vi "Sim_Check_Completion.vi"(9 "State":T3=enum."CHARGING", 10 "Settings":T4={"UI Update Interval (ms)"=200, "Max dt (s)"=1.0, "Initial SOC (%)"=50.0, "Rest Voltage (V)"=12.0, "Ambient Temperature (degC)"=25.0, "Voltage Time Constant (s)"=5.0, "Current Time Constant (s)"=1.0, "Thermal Time Constant (s)"=120.0, "Heating Coefficient (degC/s per A^2)"=0.002, "SOC Speed Factor"=1.0, "Charge Complete SOC (%)"=100.0, "Discharge Complete SOC (%)"=0.0, "Max Voltage Limit (V)"=15.0, "Max Current Limit (A)"=10.0, "Max Temperature Limit (degC)"=45.0, "Max C-Rate (1/h)"=5.0, "Max Duration (min)"=600.0, "History Length (samples)"=3000, "Inject E-Stop"=FALSE, "Inject Overvoltage"=FALSE, "Inject Overcurrent"=FALSE, "Inject Overtemperature"=FALSE}, 11 "Sim Data in":T1) -> (2 "Done?":bool, 3 "Sim Data out":T1)   [LabVIEW 2019]
doc: "Completion check for CHARGING / DISCHARGING. Done when the SOC target is reached (charge: SOC at or above Charge Complete SOC; discharge: SOC at or below Discharge Complete SOC) or the setpoint duration has elapsed. CYCLE DEFINITION: a half-cycle counts only when its SOC target is reached; duration expiry does not count. When both halves are done (either order) Cycle Count increments once and both flags clear. Not done: data passes through unchanged."
uses:
  Sim_Data.ctl
  Test_State_Enum2.ctl
  Sim_Settings.ctl
  Sim_State_Enum.ctl
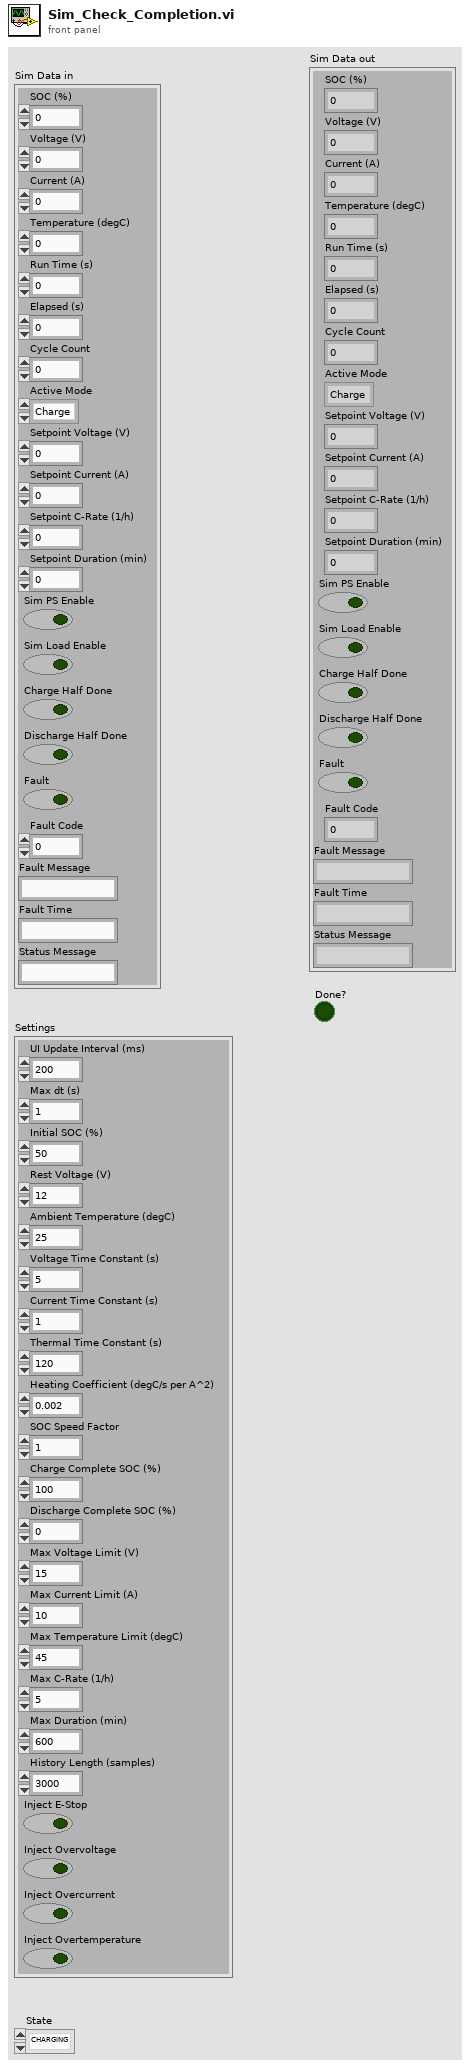
[diagram p1: front panel]
types:
  T1 = typedef "Sim_Data.ctl" = cluster{"SOC (%)":dbl, "Voltage (V)":dbl, "Current (A)":dbl, "Temperature (degC)":dbl, "Run Time (s)":dbl, "Elapsed (s)":dbl, "Cycle Count":u32, "Active Mode":T2, "Setpoint Voltage (V)":dbl, "Setpoint Current (A)":dbl, "Setpoint C-Rate (1/h)":dbl, "Setpoint Duration (min)":dbl, "Sim PS Enable":bool, "Sim Load Enable":bool, "Charge Half Done":bool, "Discharge Half Done":bool, "Fault":bool, "Fault Code":i32, "Fault Message":string, "Fault Time":string, "Status Message":string}
  T2 = typedef "Test_State_Enum2.ctl" = enum16{"Charge", "Discharge"}
  T3 = typedef "Sim_State_Enum.ctl" = enum16{"INIT", "IDLE", "CHARGING", "DISCHARGING", "STOPPED", "FAULT"}
  T4 = typedef "Sim_Settings.ctl" = cluster{"UI Update Interval (ms)":i32, "Max dt (s)":dbl, "Initial SOC (%)":dbl, "Rest Voltage (V)":dbl, "Ambient Temperature (degC)":dbl, "Voltage Time Constant (s)":dbl, "Current Time Constant (s)":dbl, "Thermal Time Constant (s)":dbl, "Heating Coefficient (degC/s per A^2)":dbl, "SOC Speed Factor":dbl, "Charge Complete SOC (%)":dbl, "Discharge Complete SOC (%)":dbl, "Max Voltage Limit (V)":dbl, "Max Current Limit (A)":dbl, "Max Temperature Limit (degC)":dbl, "Max C-Rate (1/h)":dbl, "Max Duration (min)":dbl, "History Length (samples)":i32, "Inject E-Stop":bool, "Inject Overvoltage":bool, "Inject Overcurrent":bool, "Inject Overtemperature":bool}
  T5 = enum16{"INIT", "IDLE", "CHARGING", "DISCHARGING", "STOPPED", "FAULT"}
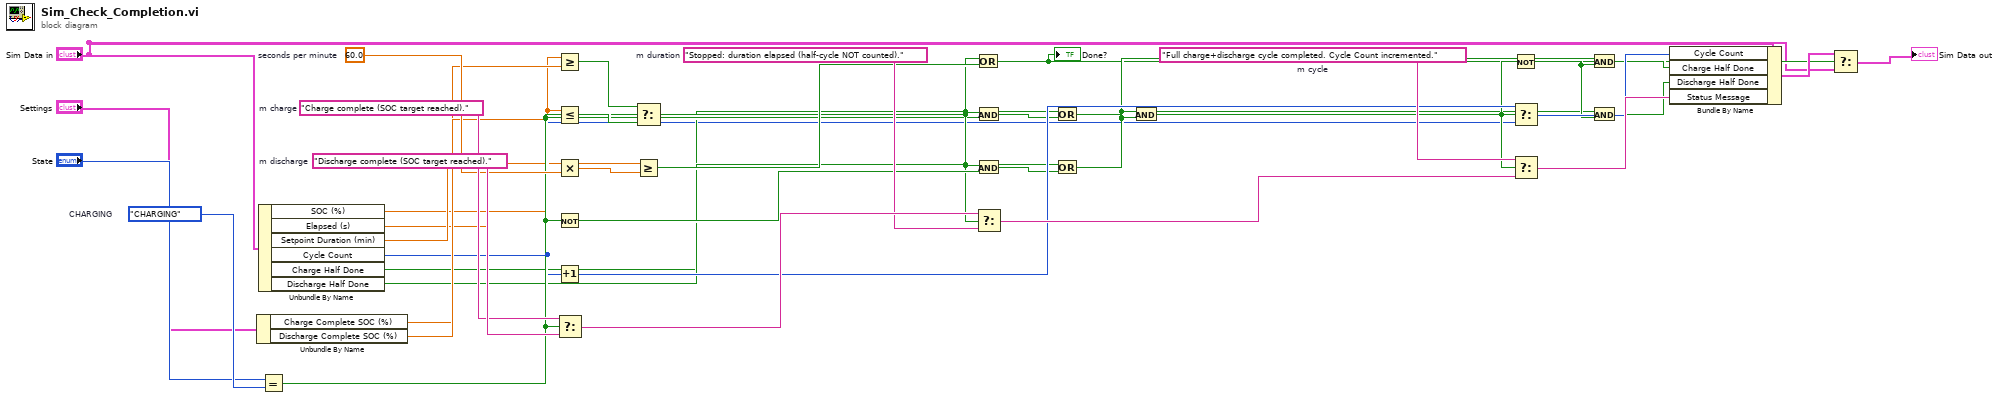
[diagram p0: block diagram]
diagram:
  w36 = "Full charge+discharge cycle completed. Cycle Count incremented."  # m cycle
  w35 = "Stopped: duration elapsed (half-cycle NOT counted)."  # m duration
  w34 = "Discharge complete (SOC target reached)."  # m discharge
  w33 = "Charge complete (SOC target reached)."  # m charge
  w19 = 60.0  # seconds per minute
  w14 = T5."CHARGING"  # CHARGING
  n1 = Unbundle By Name("Settings") -> ("Charge Complete SOC (%)"=w12:dbl, "Discharge Complete SOC (%)"=w13:dbl)
  n2 = Unbundle By Name("Sim Data in") -> ("SOC (%)"=w6:dbl, "Elapsed (s)"=w7:dbl, "Setpoint Duration (min)"=w8:dbl, "Cycle Count"=w9:u32, "Charge Half Done"=w10:bool, "Discharge Half Done"=w11:bool)
  n3 = Equal?(x="State", y=w14) -> (x = y?=w15:bool)
  n4 = Greater Or Equal?(x=w6, y=w12) -> (x >= y?=w16:bool)
  n5 = Less Or Equal?(x=w6, y=w13) -> (x <= y?=w17:bool)
  n6 = Multiply(x=w8, y=w19) -> (x*y=w20:dbl)
  n7 = Not(x=w15) -> (.not. x?=w22:bool)
  n8 = Increment(x=w9) -> (x+1=w31:u32)
  n9 = Select(t=w33, s=w15, f=w34) -> (s? t:f=w37:string)
  n10 = Select(t=w16, s=w15, f=w17) -> (s? t:f=w18:bool)
  n11 = Greater Or Equal?(x=w7, y=w20) -> (x >= y?=w21:bool)
  n12 = Or(x=w18, y=w21) -> (x .or. y?=w5:bool)
  "Done?" <- w5
  n13 = And(x=w18, y=w15) -> (x .and. y?=w23:bool)
  n14 = And(x=w18, y=w22) -> (x .and. y?=w24:bool)
  n15 = Select(t=w37, s=w18, f=w35) -> (s? t:f=w38:string)
  n16 = Or(x=w10, y=w23) -> (x .or. y?=w25:bool)
  n17 = Or(x=w11, y=w24) -> (x .or. y?=w26:bool)
  n18 = And(x=w25, y=w26) -> (x .and. y?=w27:bool)
  n19 = Not(x=w27) -> (.not. x?=w28:bool)
  n20 = Select(t=w31, s=w27, f=w9) -> (s? t:f=w32:u32)
  n21 = Select(t=w36, s=w27, f=w38) -> (s? t:f=w39:string)
  n22 = And(x=w25, y=w28) -> (x .and. y?=w29:bool)
  n23 = And(x=w26, y=w28) -> (x .and. y?=w30:bool)
  n24 = Bundle By Name(cluster="Sim Data in", "Cycle Count"=w32, "Charge Half Done"=w29, "Discharge Half Done"=w30, "Status Message"=w39) -> (w40:T1)
  n25 = Select(t=w40, s=w5, f="Sim Data in") -> (s? t:f=→"Sim Data out":T1)
